vi "Global-services.vi"() -> ()   [LabVIEW 2020, in "Sgraph_lib_V1.lvlib"]
uses:
  Builds/Sgraph_lib_V1.lvlib
panel:
  in  "DBAL-service":refnum<vi>
  in  "Gserver-service":refnum<vi>
  in  "HISW-service":refnum<vi>
  in  "FAMM-service":refnum<vi>
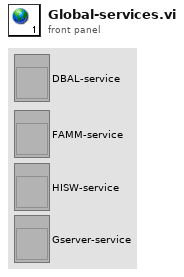
[diagram p1: front panel]
diagram:
